vi "Com_detect.vi"(10 "working directory":path=path "D:/ONGOING/EMLINQ/Emlinq_Small_Sensor_Board_Test_Software/Emlinq_Small_Sensor_Board_Test_Software/LabVIEW Files/support/com_detection") -> (2 "Barcode":refnum<visa-resource-name>, 3 "HIPOT":refnum<visa-resource-name>, 4 "Array 3":string[](array[string]))   [LabVIEW 2021]
panel:
  out "concatenated string":string
  out "standard output":string
  out "error out":errorcluster
  in  "error in":errorcluster
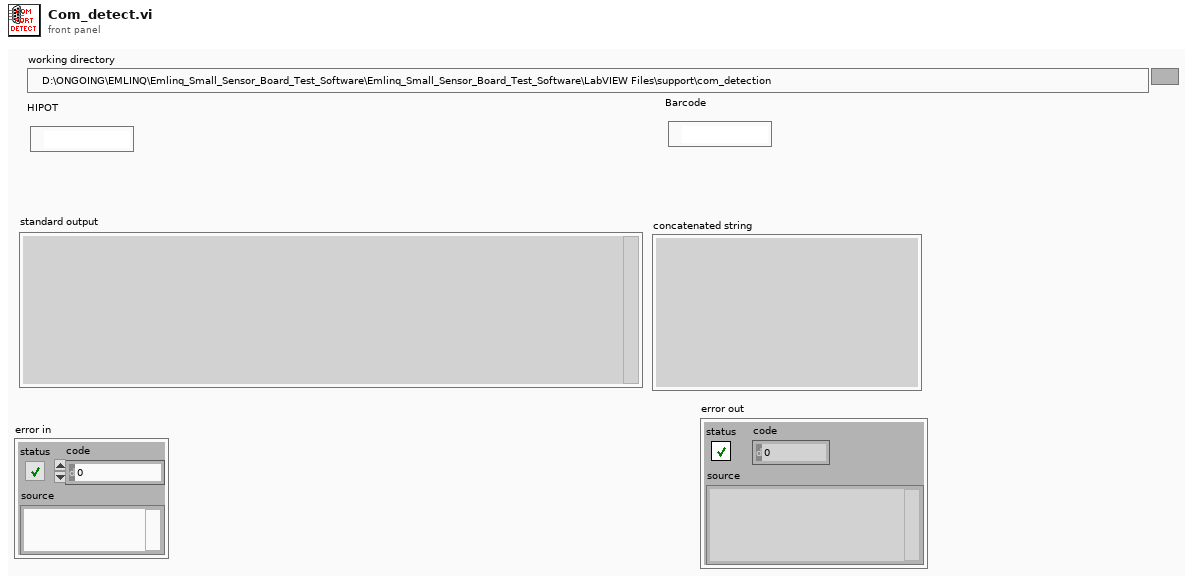
[diagram p1: front panel]
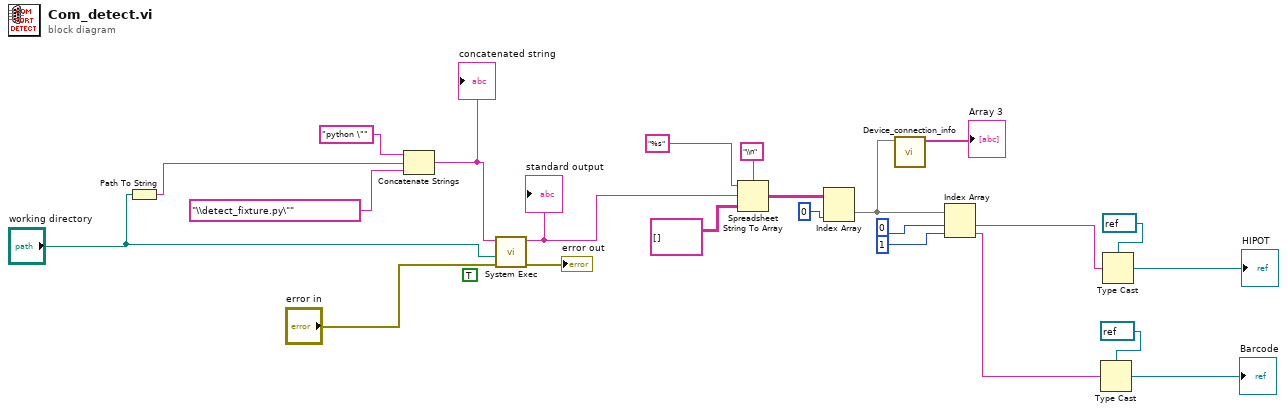
[diagram p0: block diagram]
diagram:
  (unwired) TRUE ("run minimized?")
  n1 = Path To String(path="working directory") -> (string=w11:string)
  n2 = Concatenate Strings("python \"" ("string"), w11, "\\detect_fixture.py\"" ("command line")) -> (w5:string)
  "concatenated string" <- w5
  n3 = call <vilib>:"System Exec.vi"("error in (no error)"="error in", "working directory"="working directory", "command line"=w5) -> ("error out"=→"error out":errorcluster, "standard output"=w6:string)  [unwired: 5 in, 2 out]
  "standard output" <- w6
  n4 = Spreadsheet String To Array(delimiter (Tab)="\\n", format string="%s" ("delimiter (Tab)"), spreadsheet string=w6, array type (2D Dbl)=string[][] []) -> (array=w18:string[][])
  n5 = Index Array(array=w18, index (col)=0 ("disabled index (col)")) -> (element=w13:string[])  [unwired: 1 in]
  n6 = call "Device_connection_info.vi"("Array"=w13) -> ("Array 3"=→"Array 3":string[])  [unwired: 10 in]
  n7 = Index Array(array=w13, index #1=0 ("index"), index #2=1 ("index")) -> (element #1=w14:string, element #2=w1:string)
  n8 = Type Cast(type=refnum<visa-resource-name> refnum ("Resource Name"), x=w1) -> (*(type *) &x=→"Barcode":refnum<visa-resource-name>)
  n9 = Type Cast(type=refnum<visa-resource-name> refnum ("Resource Name"), x=w14) -> (*(type *) &x=→"HIPOT":refnum<visa-resource-name>)
